vi "Handle Message.vi"(8 "error in (no error)":errorcluster, 9 "Message Completion Handler":refnum<class "Message Completion Handler.lvclass">, 10 "Message":string, 11 "Nominal-TDMS-Upload in":refnum<class "Nominal-TDMS-Upload.lvclass">) -> (0 "error out":errorcluster, 1 "Synchronously Complete Message?":bool=TRUE, 2 "Message Response":string, 3 "Nominal-TDMS-Upload out":refnum<class "Nominal-TDMS-Upload.lvclass">)   [LabVIEW 2020, in "Nominal-TDMS-Upload.lvlib" / "Nominal-TDMS-Upload.lvclass"]
uses:
  Nominal-TDMS-Upload.lvclass
  <vilib>/FlexLogger/SDK/PluginSDK.lvlibp/PEFClasses/SDK/Message Completion Handler/Message Completion Handler.lvclass
  Nominal-TDMS-Upload.lvclass/Nominal-TDMS-Upload.ctl
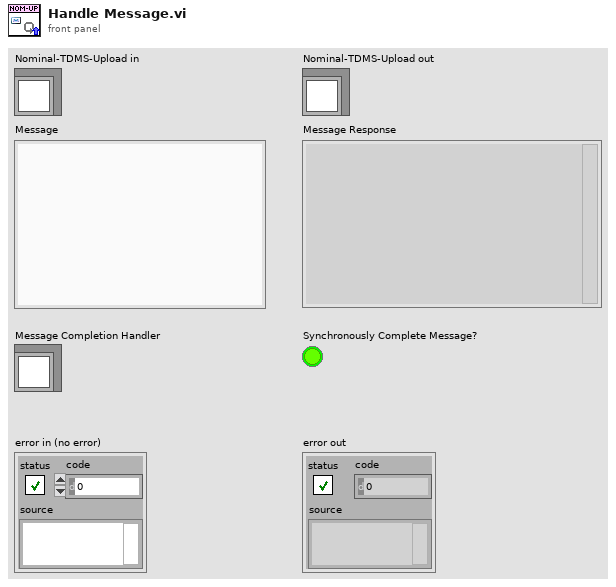
[diagram p1: front panel]
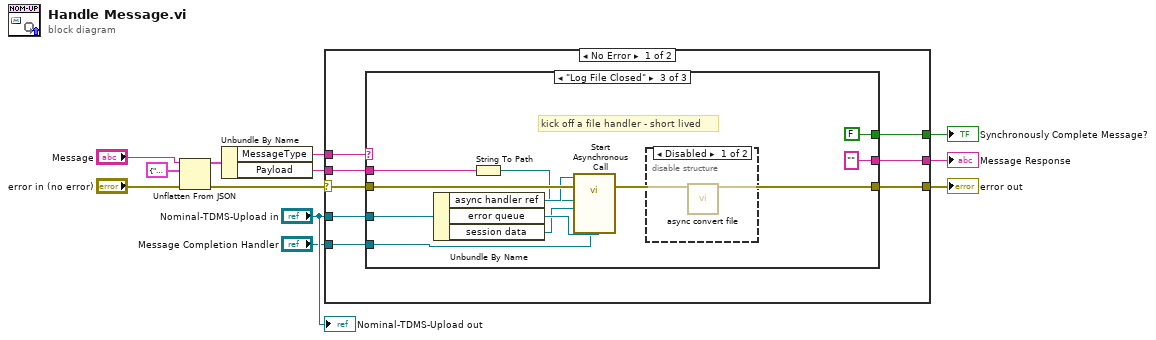
[diagram p0: block diagram]
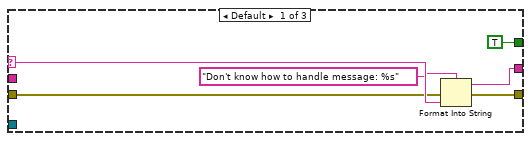
[diagram p2: hidden frame]
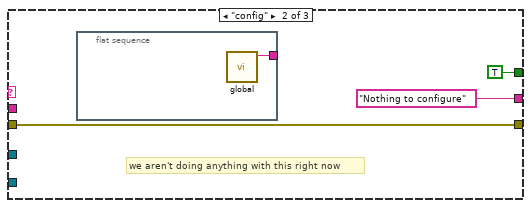
[diagram p3: hidden frame]
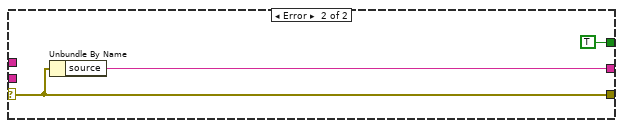
[diagram p5: hidden frame]
diagram:
  n1 = Unflatten From JSON(JSON string="Message", type and defaults=cluster{"Payload":string, "MessageType":string} {"Payload"="", "MessageType"=""}, error in (no error)="error in (no error)") -> (value=w9:cluster{"Payload":string, "MessageType":string}, error out=w8:errorcluster)  [unwired: 4 in]
  n2 = Unbundle By Name(w9) -> ("MessageType"=w6:string, "Payload"=w1:string)
  n3 = case shown="No Error" w8 {
    selector: w8 -> [w17 w44]
    tunnel: [w16 w44] -> w7
    tunnel: w6 -> [w20 _]
    tunnel: [w19 w43] -> w5
    tunnel: [w18 TRUE] -> w4
    tunnel: "Nominal-TDMS-Upload in" -> [w15 _]
    tunnel: "Message Completion Handler" -> [w14 _]
    tunnel: w1 -> [w13 _]
    frame No Error {
      n4 = case shown="\"Log File Closed\"" w20 {
        selector: w20 -> [w26 _ _]
        tunnel: [w25 "Nothing to configure" ""] -> w19
        tunnel: [TRUE TRUE FALSE] -> w18
        tunnel: w17 -> [w23 w28 w39]
        tunnel: [w22 w28 w37] -> w16
        tunnel: w15 -> [_ _ w38]
        tunnel: w14 -> [_ _ w34]
        tunnel: w13 -> [_ _ w33]
        frame Default {
          n5 = Format Into String(format string="Don't know how to handle message: %s", error in=w23, w26) -> (resulting string=w25:string, error out=w22:errorcluster)  [unwired: 1 in]
        }
        frame "config" {
          # "we aren't doing anything with this right now"
          n6 = flat-sequence {
            tunnel: [w30] -> _
            frame #0 {
              n7 = call "global.vi"() -> ("command"=w30:string)  [unwired: 9 in, 2 out]
            }
          }
        }
        frame "Log File Closed" {
          # "kick off a file handler - short lived"
          n8 = Unbundle By Name(w38) -> ("async handler ref"=w36:refnum<vi>, "error queue"=w35:refnum<queue>, "session data"=w31:refnum<data-value>)
          n9 = String To Path(string=w33) -> (path=w32:path)
          n10 = call-by-ref "Start Asynchronous Call"(reference=w36, error in=w39, "error queue"=w35, "Message Completion Handler"=w34, "session data"=w31, "TDMS File"=w32) -> (error out=w37:errorcluster)  [unwired: 8 in, 1 out]
          n11 = disable-structure shown="Disabled" {
            frame Disabled {
              n12 = call "async convert file.vi"() -> ()  [unwired: 12 in]
            }
            frame Enabled {
            }
          }
        }
      }
    }
    frame Error {
      n13 = Unbundle By Name(w44) -> ("source"=w43:string)
    }
  }
  "error out" <- w7
  "Message Response" <- w5
  "Synchronously Complete Message?" <- w4
  "Nominal-TDMS-Upload out" <- "Nominal-TDMS-Upload in"
